vi "FuncVI-Polar.vi"(5 "InstanceRef":T2, 9 "arg list":T1[](array[typedef]) {"num" format="%.2f"}) -> (0 "error out":bool, 3 "result":T1 {"num" format="%.2f"})   [LabVIEW 2021]
doc: "::: CalcExpress Toolkit :::\nCopyright (c) 2000-2026 Konstantin Shifershteyn. All rights reserved."
uses:
  cetypes.llb/CalcExpress Function Argument Info.ctl
  cetypes.llb/CalcExpress Instance RefNum.ctl
panel:
  in  "max arg num":i32=2
  in  "min arg num":i32=1
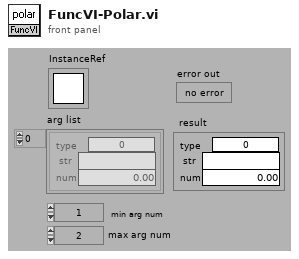
[diagram p1: front panel]
types:
  T1 = typedef "CalcExpress Function Argument Info.ctl" = cluster{"type":u32, "str":string, "num":dbl}
  T2 = typedef "CalcExpress Instance RefNum.ctl" = refnum<k1>
  T3 = enum16{"Array-Array", "Array-Scalar", "Scalar-Array", "Scalar-Scalar"}
  T4 = cluster{"Left 2D":cdb[][], "Left Scalar":cdb, "Right 2D":cdb[][], "Right Scalar":cdb}
  T5 = cluster{"Left 2D":dbl[][], "Left Scalar":dbl, "Right 2D":dbl[][], "Right Scalar":dbl}
  T6 = typedef "CalcExpress Data Type.ctl" = enum32{"String", "DBL Number", "identifier", "1D Array of DBL", "2D Array of DBL", "CDB Number", "1D Array of CDB", "2D Array of CDB", "1D Array of String", "2D Array of String", "Unknown data type"}
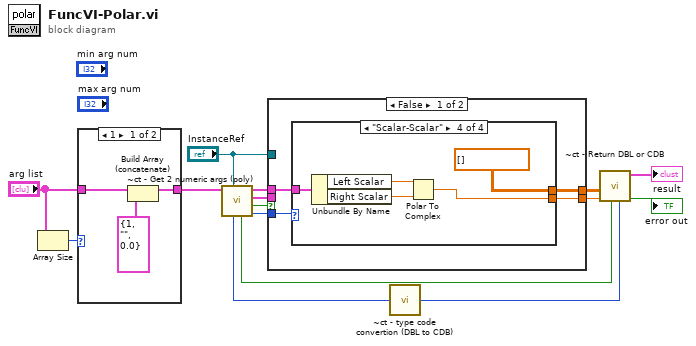
[diagram p0: block diagram]
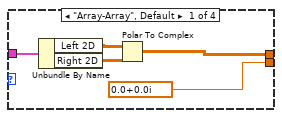
[diagram p3: hidden frame]
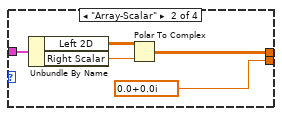
[diagram p4: hidden frame]
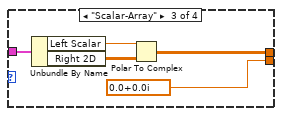
[diagram p5: hidden frame]
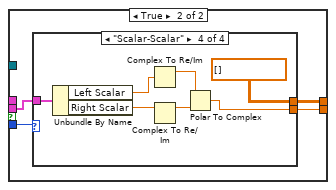
[diagram p6: hidden frame]
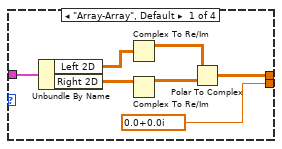
[diagram p7: hidden frame]
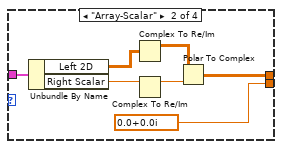
[diagram p8: hidden frame]
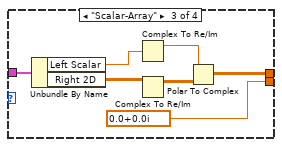
[diagram p9: hidden frame]
diagram:
  n1 = Array Size(array="arg list") -> (size(s)=w7:i32)
  n2 = case shown="1" w7 {
    tunnel: "arg list" -> [w18 w19]
    tunnel: [w17 w19] -> w5
    frame 1 {
      n3 = Build Array (concatenate)(w18, cluster{"type":u8, "str":string, "num":dbl} {"type"=1, "str"="", "num"=0.0} ("arg info")) -> (w17:T1[])
    }
    frame 2, Default {
    }
  }
  n4 = call "~ct - Get 2 numeric args (poly).vi"("InstanceRef"="InstanceRef", "args list"=w5) -> ("poly"=w9:T3, "CDB ?"=w12:bool, "CDB arguments"=w10:T4, "DBL arguments"=w11:T5, "error out"=w4:bool, "type of result"=w13:T6)  [unwired: 4 in]
  n5 = case shown="False" w12 {
    tunnel: w11 -> [w22 _]
    tunnel: w10 -> [_ w44]
    tunnel: w9 -> [w23 w47]
    tunnel: [w21 w46] -> w1
    tunnel: [w20 w45] -> w2
    tunnel: "InstanceRef" -> [_ _]
    frame False {
      n6 = case shown="\"Scalar-Scalar\"" w23 {
        tunnel: w22 -> [w28 w33 w38 w43]
        tunnel: [w24 w29 w34 cdb[][] []] -> w21
        tunnel: [cdb 0.0+0.0i cdb 0.0+0.0i cdb 0.0+0.0i w39] -> w20
        frame "Array-Array", Default {
          n7 = Unbundle By Name(w28) -> ("Left 2D"=w26:dbl[][], "Right 2D"=w25:dbl[][])
          n8 = Polar To Complex(1:w25, 2:w26) -> (0:w24:cdb[][])
        }
        frame "Array-Scalar" {
          n9 = Unbundle By Name(w33) -> ("Left 2D"=w31:dbl[][], "Right Scalar"=w30:dbl)
          n10 = Polar To Complex(1:w30, 2:w31) -> (0:w29:cdb[][])
        }
        frame "Scalar-Array" {
          n11 = Unbundle By Name(w38) -> ("Left Scalar"=w36:dbl, "Right 2D"=w35:dbl[][])
          n12 = Polar To Complex(1:w35, 2:w36) -> (0:w34:cdb[][])
        }
        frame "Scalar-Scalar" {
          n13 = Unbundle By Name(w43) -> ("Left Scalar"=w41:dbl, "Right Scalar"=w40:dbl)
          n14 = Polar To Complex(1:w40, 2:w41) -> (0:w39:cdb)
        }
      }
    }
    frame True {
      n15 = case shown="\"Scalar-Scalar\"" w47 {
        tunnel: w44 -> [w54 w61 w68 w75]
        tunnel: [w52 w59 w66 cdb[][] []] -> w46
        tunnel: [cdb 0.0+0.0i cdb 0.0+0.0i cdb 0.0+0.0i w73] -> w45
        frame "Array-Array", Default {
          n16 = Unbundle By Name(w54) -> ("Left 2D"=w49:cdb[][], "Right 2D"=w50:cdb[][])
          n17 = Complex To Re/Im(x + iy=w49) -> (x=w48:dbl[][])  [unwired: 1 out]
          n18 = Complex To Re/Im(x + iy=w50) -> (x=w51:dbl[][])  [unwired: 1 out]
          n19 = Polar To Complex(1:w51, 2:w48) -> (0:w52:cdb[][])
        }
        frame "Array-Scalar" {
          n20 = Unbundle By Name(w61) -> ("Left 2D"=w56:cdb[][], "Right Scalar"=w58:cdb)
          n21 = Complex To Re/Im(x + iy=w56) -> (x=w55:dbl[][])  [unwired: 1 out]
          n22 = Complex To Re/Im(x + iy=w58) -> (x=w57:dbl)  [unwired: 1 out]
          n23 = Polar To Complex(1:w57, 2:w55) -> (0:w59:cdb[][])
        }
        frame "Scalar-Array" {
          n24 = Unbundle By Name(w68) -> ("Left Scalar"=w63:cdb, "Right 2D"=w65:cdb[][])
          n25 = Complex To Re/Im(x + iy=w63) -> (x=w62:dbl)  [unwired: 1 out]
          n26 = Complex To Re/Im(x + iy=w65) -> (x=w64:dbl[][])  [unwired: 1 out]
          n27 = Polar To Complex(1:w64, 2:w62) -> (0:w66:cdb[][])
        }
        frame "Scalar-Scalar" {
          n28 = Unbundle By Name(w75) -> ("Left Scalar"=w70:cdb, "Right Scalar"=w72:cdb)
          n29 = Complex To Re/Im(x + iy=w70) -> (x=w69:dbl)  [unwired: 1 out]
          n30 = Complex To Re/Im(x + iy=w72) -> (x=w71:dbl)  [unwired: 1 out]
          n31 = Polar To Complex(1:w71, 2:w69) -> (0:w73:cdb)
        }
      }
    }
  }
  n32 = call "~ct - type code convertion (DBL to CDB).vi"("type"=w13) -> ("type out"=w3:T6)  [unwired: 4 in]
  n33 = call "~ct - Return DBL or CDB.vi"("type"=w3, "error in"=w4, "CDB"=w2, "2D CDB"=w1) -> ("error out"=→"error out":bool, "result"=→"result":T1)  [unwired: 6 in]
